vi "Extract Sector and Image From Binary.vi"(0 "Binary Data(u64)":u64[](array[numeric]), 1 "Start Index":u64, 5 "# of u64 per image":u64, 7 "Height":i32, 9 "Width":i32, 11 "error in (no error)":errorcluster, 12 "Image Destination":T1) -> (4 "Image Out":T1, 6 "Left Sector":u16, 8 "Right Sector":u16, 10 "Log?":bool, 15 "error out":errorcluster)   [LabVIEW 2013]
uses:
  <vilib>/vision/Image Controls.llb/IMAQ Image.ctl
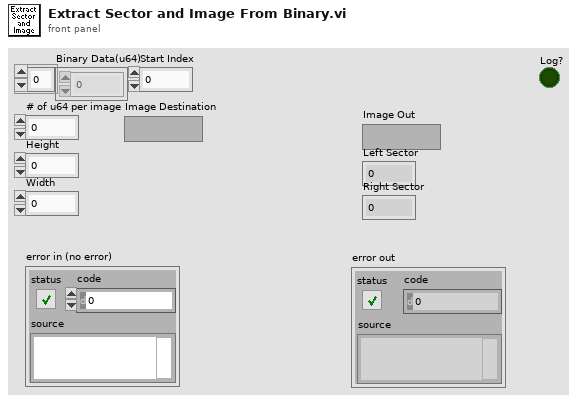
[diagram p1: front panel]
types:
  T1 = typedef "IMAQ Image.ctl" = refnum<image>
  T2 = enum16{"big-endian, network order", "native, host order", "little-endian"}
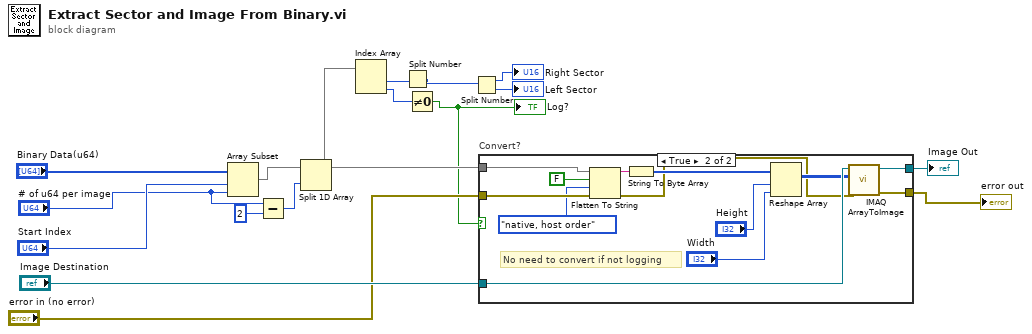
[diagram p0: block diagram]
diagram:
  n1 = Array Subset(array="Binary Data(u64)", index="Start Index", length="# of u64 per image") -> (w17:u64[])
  n2 = Subtract(x="# of u64 per image", y=u64 2) -> (x-y=w4:u64)
  n3 = Split 1D Array(array=w17, index=w4) -> (first subarray=w3:u64[], second subarray=w2:u64[])
  n4 = Index Array(array=w2) -> (element #1=w14:u64, element #2=w5:u64)  [unwired: 2 in]
  n5 = Split Number(x=w14) -> (lo(x)=w13:u32)  [unwired: 1 out]
  n6 = Not Equal To 0?(x=w5) -> (x != 0?=w1:bool)
  "Log?" <- w1
  n7 = Split Number(x=w13) -> (hi(x)=→"Right Sector":u16, lo(x)=→"Left Sector":u16)
  n8 = case "Convert?" shown="True" w1 {
    tunnel: "Image Destination" -> [w20 w33]
    tunnel: [w20 w30] -> w15
    tunnel: "error in (no error)" -> [w19 w27]
    tunnel: [w19 w22] -> w9
    tunnel: w3 -> [_ w21]
    frame False {
    }
    frame True {
      # "No need to convert if not logging"
      n9 = Flatten To String(anything=w21, prepend array or string size? (T)=FALSE, byte order (0:big-endian, network order)=T2."native, host order", error in (no error)=w27) -> (data string=w23:string, error out=w26:errorcluster)  [unwired: 1 out]
      n10 = String To Byte Array(string=w23) -> (unsigned byte array=w32:u8[])
      n11 = Reshape Array(w32, "Height", "Width") -> (w31:u8[][])
      n12 = call "IMAQ ArrayToImage"("error in (no error)"=w26, "Image Pixels (U8)"=w31, "Image"=w33) -> ("error out"=w22:errorcluster, "Image Out"=w30:T1)  [unwired: 7 in]
    }
  }
  "error out" <- w9
  "Image Out" <- w15
